vi "Set Activation Arguments.vi"(8 "error in (no error)":errorcluster, 10 "launchArgs":string, 11 "ToastBuilder in":refnum<class "ToastBuilder.lvclass">) -> (0 "error out":errorcluster, 3 "ToastBuilder out":refnum<class "ToastBuilder.lvclass">)   [LabVIEW 2026, in "ToastNotification.lvlib" / "ToastBuilder.lvclass"]
doc: "Sets the raw arguments returned when the notification body is clicked. Uses the encapsulated builder with Foreground activation. launchArgs replaces the previous body launch string and is passed through unchanged; the method does not parse or encode key/value pairs. Button arguments remain configured by the button methods. Call after Create and before Show. An incoming error passes the input class and error through unchanged. No .NET reference is exposed or closed; builder ownership remains with the caller. Activation arguments are distinct from submitted User Inputs."
uses:
  ToastBuilder.lvclass
  ToastBuilder.lvclass/ToastBuilder.ctl
  Read Builder Reference.vi
  Write Builder Reference.vi
  Toast Native/Toast Native.lvlib
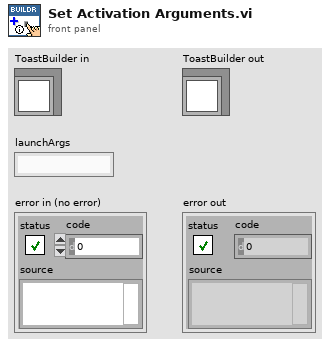
[diagram p1: front panel]
types:
  T1 = typedef "ToastNotification.lvlib/ToastBuilder.lvclass/Builder Reference.ctl" = refnum<k24>
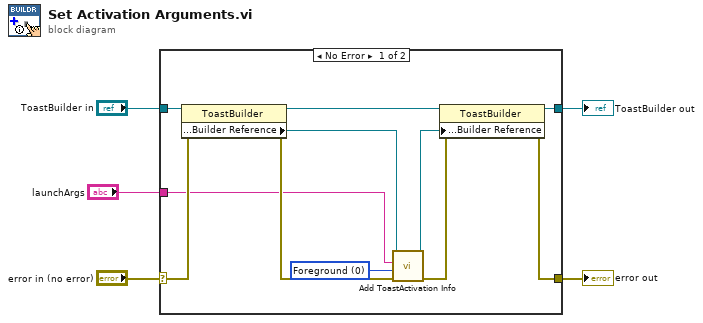
[diagram p0: block diagram]
diagram:
  n1 = case shown="No Error" "error in (no error)" {
    selector: "error in (no error)" -> [w13 w18]
    tunnel: [w12 w18] -> w4
    tunnel: [w14 w17] -> w2
    tunnel: "ToastBuilder in" -> [w16 w17]
    tunnel: "launchArgs" -> [w7 _]
    frame No Error {
      w6 = 0 items=["Foreground", "Background", "Protocol"] ("activationType")
      n2 = property class="ToastBuilder"(reference=w16, error in=w13) -> (reference out=w15:refnum<class "ToastBuilder.lvclass">, error out=w11:errorcluster, "Public:Properties:Builder Reference"=w9:T1)
      n3 = call "Add ToastActivation Info.vi"("error in (no error)"=w11, "activationType"=w6, "launchArgs"=w7, "reference"=w9) -> ("error out"=w10:errorcluster, "reference out"=w8:refnum<k24>)  [unwired: 6 in]
      n4 = property class="ToastBuilder"(reference=w15, error in=w10, "Public:Properties:Builder Reference"=w8) -> (reference out=w14:refnum<class "ToastBuilder.lvclass">, error out=w12:errorcluster)
    }
    frame Error {
    }
  }
  "error out" <- w4
  "ToastBuilder out" <- w2
